vi "RemoteVI Tips Message.vi"(0 "tips":T1(array[cluster])) -> (4 "message":string)   [LabVIEW 2020, in "RemoteVI.lvlib"]
doc: "Builds the text message tips <json> (docs\\protocol.md section 3.3) from the tip strips RemoteVI Read Tips.vi read: a JSON array with one object per control whose tip strip text is not empty, x, y, w, h, text in that order - tips [] when there is none. text is the control's Tip Strip as LabVIEW holds it (bytes of the system code page); each byte is widened to one UTF-16 code unit (exact for ASCII and Latin-1; Windows-1252 differs only in 0x80-0x9F) and written as an ASCII-only JSON string literal by RemoteVI JSON String.vi, so the message is valid UTF-8 whatever the host's code page. The JSON is written field by field, like RemoteVI Windows Message.vi. Pure function, cannot fail. Reference: tipsMessage() in tools\\lib\\protocol.mjs, vectors tests\\vectors\\text.json."
uses:
  RemoteVI.lvlib
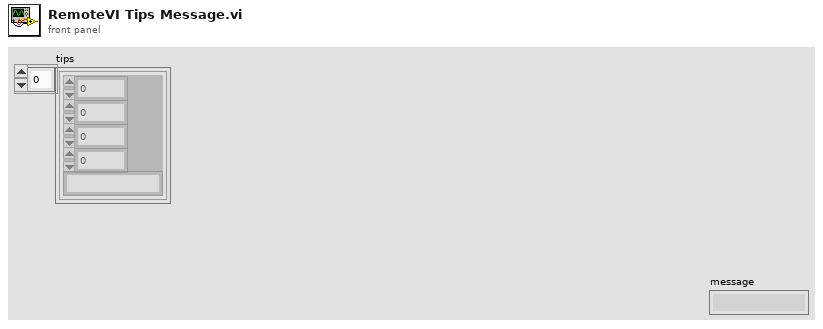
[diagram p1: front panel]
types:
  T1 = cluster{"x":i32, "y":i32, "w":i32, "h":i32, "text":string}[]
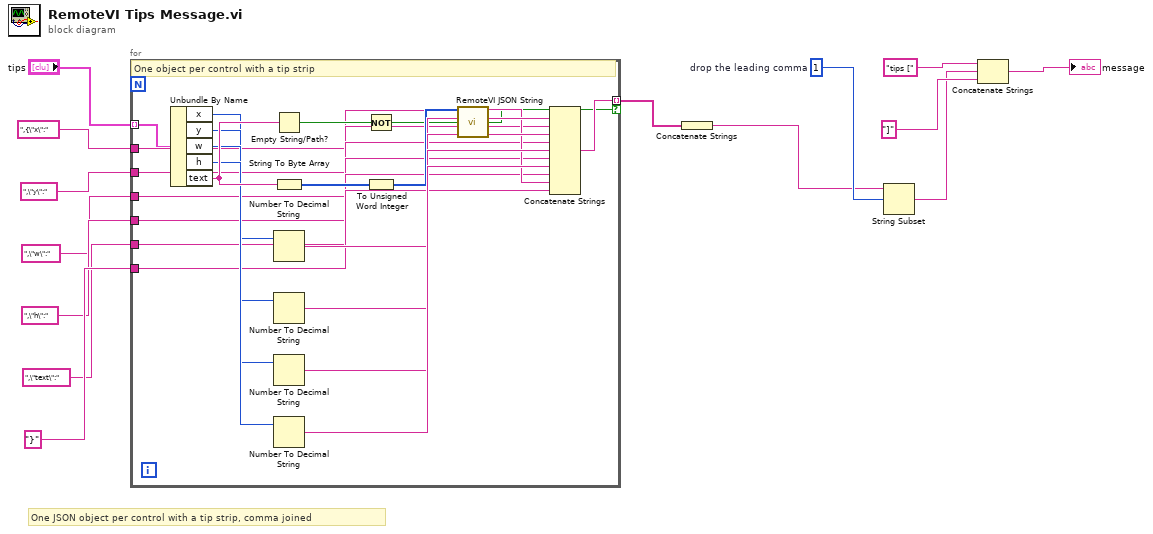
[diagram p0: block diagram]
diagram:
  w10 = 1  # drop the leading comma
  # "One JSON object per control with a tip strip, comma joined"
  n1 = for {
    tunnel: "tips" -> [w15] mode=indexing
    tunnel: ",{\"x\":" -> [w16]
    tunnel: ",\"y\":" -> [w17]
    tunnel: ",\"w\":" -> [w18]
    tunnel: ",\"h\":" -> [w19]
    tunnel: ",\"text\":" -> [w20]
    tunnel: "}" -> [w21]
    tunnel: [w36] -> w8 mode=indexing if=w28
    # "One object per control with a tip strip"
    n2 = Unbundle By Name(w15) -> ("x"=w22:i32, "y"=w23:i32, "w"=w24:i32, "h"=w25:i32, "text"=w26:string)
    n3 = Empty String/Path?(string/path=w26) -> (empty?=w27:bool)
    n4 = String To Byte Array(string=w26) -> (unsigned byte array=w29:u8[])
    n5 = Number To Decimal String(number=w22) -> (decimal integer string=w32:string)  [unwired: 1 in]
    n6 = Number To Decimal String(number=w23) -> (decimal integer string=w33:string)  [unwired: 1 in]
    n7 = Number To Decimal String(number=w24) -> (decimal integer string=w34:string)  [unwired: 1 in]
    n8 = Number To Decimal String(number=w25) -> (decimal integer string=w35:string)  [unwired: 1 in]
    n9 = Not(x=w27) -> (.not. x?=w28:bool)
    n10 = To Unsigned Word Integer(number=w29) -> (unsigned 16bit integer=w30:u16[])
    n11 = call "RemoteVI JSON String.vi"("text"=w30) -> ("json"=w31:string)  [unwired: 14 in]
    n12 = Concatenate Strings(w16, w32, w17, w33, w18, w34, w19, w35, w20, w31, w21) -> (w36:string)
  }
  n13 = Concatenate Strings(w8) -> (w9:string)
  n14 = String Subset(string=w9, offset (0)=w10) -> (substring=w11:string)  [unwired: 1 in]
  n15 = Concatenate Strings("tips [", w11, "]") -> (→"message":string)
